vi "lvDiff.vi"   [LabVIEW 2014, in "lv-cli-steps.lvlib"]
uses:
  lv-cli-steps.lvlib
  <vilib>/Utility/error.llb/DialogType.ctl
  <vilib>/lvrevbrd/DiffVIs.lvlib
  <vilib>/Wiresmith Technology/LabVIEW CLI/CLI Class/CLI.lvclass
  <vilib>/lvrevbrd/ScreenshotVI.lvlib
types:
  T1 = typedef "DialogType.ctl" = u16
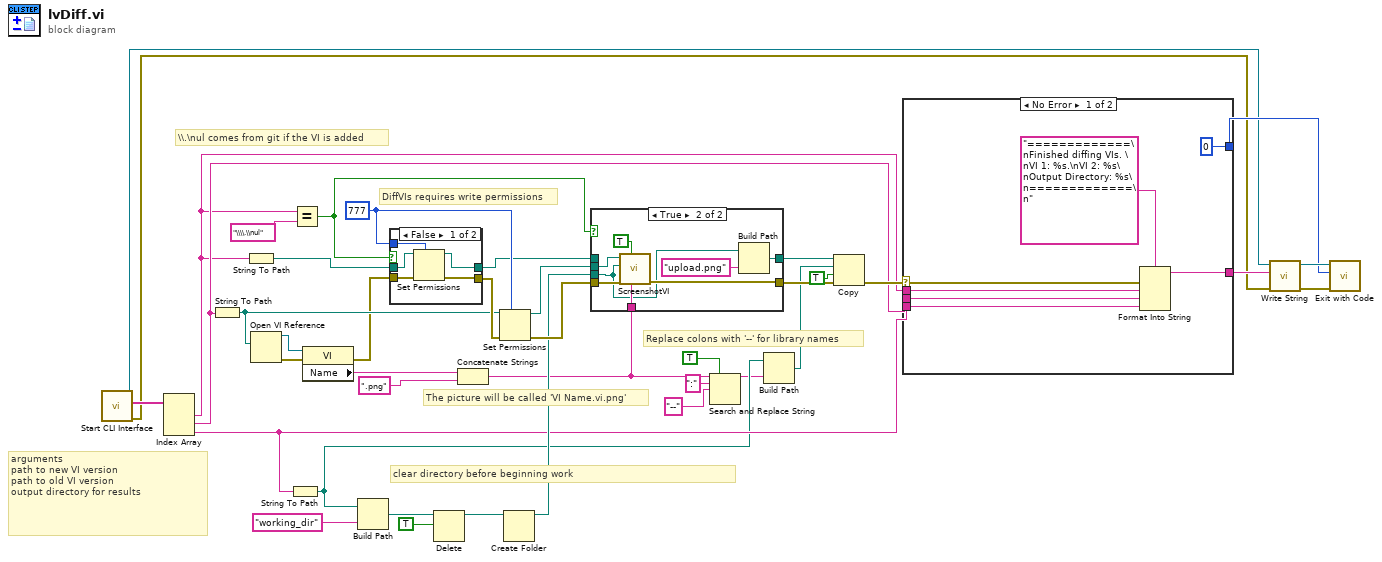
[diagram p0: block diagram]
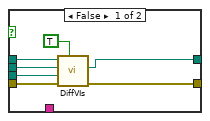
[diagram p3: hidden frame]
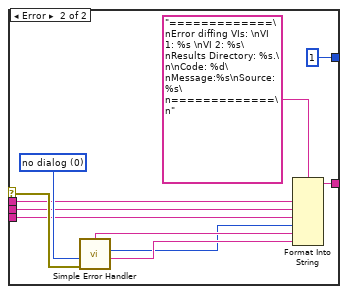
[diagram p4: hidden frame]
diagram:
  w21 = i16 777 ("permissions")
  # "\\\\.\\nul comes from git if the VI is added"
  # "Replace colons with '--' for library names"
  # "clear directory before beginning work"
  # "DiffVIs requires write permissions"
  # "The picture will be called 'VI Name.vi.png'"
  # "arguments\npath to new VI version\npath to old VI version\noutput directory for results"
  n1 = call <vilib>:"Start CLI Interface.vi"() -> ("error out"=w19:errorcluster, "Custom Parameters"=w26:string[], "CLI out"=w27:refnum<class "CLI.lvclass">)  [unwired: 9 in]
  n2 = Index Array(array=w26) -> (element #1=w5:string, element #2=w22:string, element #3=w23:string)  [unwired: 3 in]
  n3 = String To Path(string=w22) -> (path=w17:path)
  n4 = String To Path(string=w5) -> (path=w35:path)
  n5 = Open VI Reference(vi path=w17) -> (vi reference=w16:refnum<vi>, error out=w15:errorcluster)  [unwired: 5 in]
  n6 = String To Path(string=w23) -> (path=w18:path)
  n7 = Equal?(x=w5, y="\\\\.\\nul") -> (x = y?=w3:bool)
  n8 = property class="VI"(reference=w16, error in=w15) -> (error out=w14:errorcluster, "Name"=w13:string)  [unwired: 1 out]
  n9 = Build Path(base path=w18, name or relative path="working_dir") -> (appended path=w12:path)
  n10 = case shown="False" w3 {
    tunnel: w35 -> [w45 w46]
    tunnel: [w44 w47] -> w25
    tunnel: w21 -> [w43 _]
    tunnel: w14 -> [w42 w47]
    tunnel: [w41 w46] -> w2
    frame False {
      n11 = Set Permissions(7:w43, 8:w42, 11:w45) -> (0:w44:errorcluster, 3:w41:path)  [unwired: 2 in]
    }
    frame True {
    }
  }
  n12 = Delete(path (use dialog)=w12, entire hierarchy (F)=TRUE) -> (deleted path=w11:path)  [unwired: 3 in, 2 out]
  n13 = Concatenate Strings(w13, ".png" ("string")) -> (w4:string)
  n14 = Set Permissions(7:w21, 8:w25, 11:w17) -> (0:w40:errorcluster, 3:w39:path)  [unwired: 2 in]
  n15 = Create Folder(path (use dialog)=w11) -> (created path=w37:path)  [unwired: 2 in, 2 out]
  n16 = case shown="True" w3 {
    tunnel: w40 -> [w53 w59]
    tunnel: w39 -> [w52 w60]
    tunnel: [w51 w57] -> w38
    tunnel: w37 -> [w50 w55]
    tunnel: [w49 w61] -> w36
    tunnel: w4 -> [_ w58]
    tunnel: w2 -> [w48 _]
    frame False {
      n17 = call <vilib>:"DiffVIs.vi"("Take ScrShots All In"=TRUE, "error in"=w53, "Picture Save Location"=w50, "VI Path 2"=w52, "VI Path 1"=w48) -> ("error out"=w49:errorcluster, "diff file"=w51:path)  [unwired: 2 in, 3 out]
    }
    frame True {
      n18 = call <vilib>:"ScreenshotVI.vi"("Title Prefix In"=w58, "Take Scrshots All In"=TRUE, "error in"=w59, "Picture Save Location"=w55, "VI Path"=w60) -> ("error out"=w61:errorcluster)  [unwired: 3 in, 3 out]
      n19 = Build Path(base path=w55, name or relative path="upload.png") -> (appended path=w57:path)
    }
  }
  n20 = Search and Replace String(replace all?=TRUE ("replace all? (F)"), input string=w4, search string=":", replace string="--" ("replace string (\"\")")) -> (result string=w9:string)  [unwired: 4 in, 3 out]
  n21 = Build Path(base path=w18, name or relative path=w9) -> (appended path=w32:path)
  n22 = Copy(8:w36, 9:TRUE ("overwrite (F)"), 10:w32, 11:w38) -> (0:w24:errorcluster)  [unwired: 1 in, 2 out]
  n23 = case shown="No Error" w24 {
    selector: w24 -> [w68 w79]
    tunnel: [w67 w80] -> w31
    tunnel: [0 ("Exit Code (0)") 1 ("Exit Code (0)")] -> w29
    tunnel: w22 -> [w64 w71]
    tunnel: w23 -> [w63 w72]
    tunnel: w5 -> [w65 w70]
    frame No Error {
      n24 = Format Into String(format string="=============\nFinished diffing VIs. \nVI 1: %s.\nVI 2: %s\nOutput Directory: %s\n=============\n", error in=w68, w65, w64, w63) -> (resulting string=w67:string)  [unwired: 1 in, 1 out]
    }
    frame Error {
      w78 = T1 0 items=["no dialog", "OK message", "continue or stop message", "OK message + warnings", "continue/stop + warnings"] ("type of dialog (OK msg:1)")
      n25 = call <vilib>:"Simple Error Handler.vi"("type of dialog (OK msg:1)"=w78, "error in (no error)"=w79) -> ("code out"=w73:i32, "source out"=w74:string, "message"=w75:string)  [unwired: 3 in, 2 out]
      n26 = Format Into String(format string="=============\nError diffing VIs: \nVI 1: %s \nVI 2: %s\nResults Directory: %s.\n\nCode: %d\nMessage:%s\nSource: %s\n=============\n", w70, w71, w72, w73, w75, w74) -> (resulting string=w80:string)  [unwired: 2 in, 1 out]
    }
  }
  n27 = call <vilib>:"Write String.vi"("error in (no error)"=w19, "Text to Write"=w31, "CLI in"=w27) -> ("error out"=w28:errorcluster, "CLI out"=w30:refnum<class "CLI.lvclass">)  [unwired: 7 in]
  n28 = call <vilib>:"Exit with Code.vi"("error in (no error)"=w28, "Exit Code (0)"=w29, "CLI in"=w30) -> ()  [unwired: 8 in, 1 out]
